vi "Verify Cancel.vi"(7 "History":refnum<class "History.lvclass">, 11 "Calling VI":refnum<vi>) -> (0 "error out":errorcluster, 2 "Close IE":bool)   [LabVIEW 2020, in "lv_icon.lvlib"]
doc: "Checks if there were changes to the icon and allows the user to select to keep or discord those changes or to return to the Icon Editor."
uses:
  lv_icon.lvlib
  History/History/History.lvclass
panel:
  in  "Cancel":bool
  in  "Discard":bool
  in  "Apply":bool
  # "The icon has unapplied changes.\nDo you want to apply or discard the changes?"
  # "Apply the changes to the VI"
  # "Changes are discarded and the Icon Editor will be closed"
  # "Return to the Icon Editor"
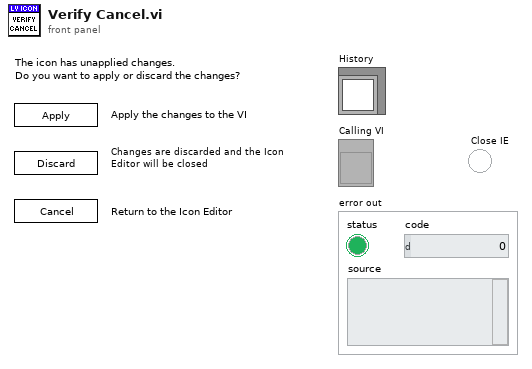
[diagram p1: front panel]
types:
  T1 = enum32{"Invalid", "Standard", "Closed", "Hidden", "Minimized", "Maximized"}
  T2 = enum32{"Invalid", "Default", "Floating", "Floating/Auto-Hide", "Modal"}
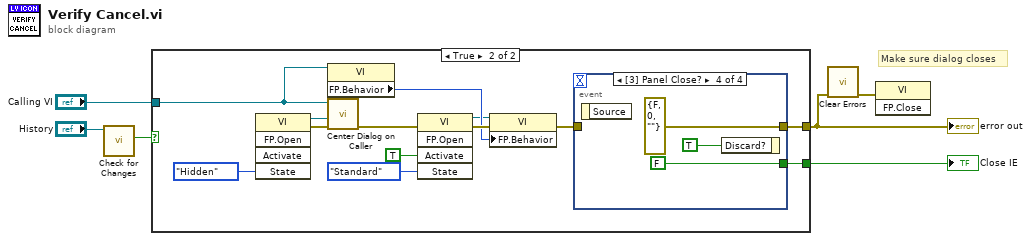
[diagram p0: block diagram]
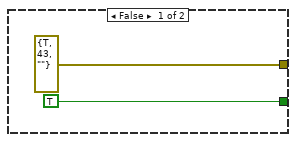
[diagram p2: hidden frame]
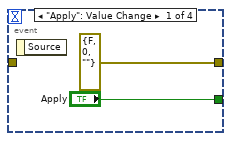
[diagram p3: hidden frame]
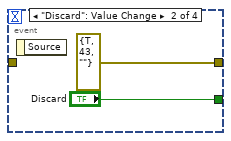
[diagram p4: hidden frame]
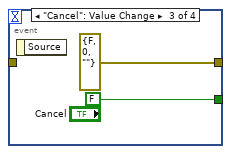
[diagram p5: hidden frame]
diagram:
  # "Make sure dialog closes"
  n1 = call "Check for Changes.vi"("History"="History") -> ("Have Changes"=w2:bool)  [unwired: 10 in]
  n2 = case shown="True" w2 {
    tunnel: [errorcluster {"status"=TRUE, "code"=43, "source"=""} ("error out") w21] -> w5
    tunnel: [TRUE ("Cancel") w15] -> w4
    tunnel: "Calling VI" -> [_ w9]
    frame False {
    }
    frame True {
      n3 = invoke class="VI" method="FP.Open"("State"=T1."Hidden") -> (reference out=w11:refnum<vi>, error out=w20:errorcluster)  [unwired: 4 in, 3 out]
      n4 = property class="VI"(reference=w9) -> ("FP.Behavior"=w16:T2)  [unwired: 1 in, 2 out]
      n5 = call "Center Dialog on Caller.vi"("error in"=w20, "Dialog VI"=w11, "Calling VI in"=w9) -> ("error out"=w19:errorcluster)  [unwired: 8 in]
      n6 = invoke class="VI" method="FP.Open"(error in=w19, "Activate"=TRUE ("Activate?"), "State"=T1."Standard") -> (reference out=w10:refnum<vi>, error out=w18:errorcluster)  [unwired: 2 in, 3 out]
      n7 = property class="VI"(reference=w10, error in=w18, "FP.Behavior"=w16) -> (error out=w17:errorcluster)  [unwired: 1 out]
      n8 = event shown="[3] Panel Close?" {
        selector: _ -> [_ _ _ _]
        dyn-events: _ -> [_ _ _ _]
        timeout: _ -> [_ _ _ _]
        tunnel: [errorcluster {"status"=FALSE, "code"=0, "source"=""} ("error out") errorcluster {"status"=TRUE, "code"=43, "source"=""} ("error out") errorcluster {"status"=FALSE, "code"=0, "source"=""} ("error out") errorcluster {"status"=FALSE, "code"=0, "source"=""} ("error out")] -> w21
        tunnel: ["Apply" "Discard" FALSE ("Discard") FALSE ("Discard")] -> w15
        tunnel: w17 -> [_ _ _ _]
        event "Apply": Value Change {
          n9 = event-data() -> ()  [unwired: 1 in, 1 out]
        }
        event "Discard": Value Change {
          n10 = event-data() -> ()  [unwired: 1 in, 1 out]
        }
        event "Cancel": Value Change {
          n11 = event-data() -> ()  [unwired: 1 in, 1 out]
        }
        event Panel Close? {
          n12 = event-data() -> ()  [unwired: 1 in, 1 out]
          n13 = event-data("Discard?"=TRUE) -> ()  [unwired: 1 in, 1 out]
        }
      }
    }
  }
  "error out" <- w5
  "Close IE" <- w4
  n14 = call <vilib>:"Clear Errors.vi"("error in (no error)"=w5) -> ("error out"=w6:errorcluster)  [unwired: 5 in, 1 out]
  n15 = invoke class="VI" method="FP.Close"(error in=w6) -> ()  [unwired: 2 in, 3 out]
